vi "Get Default Actor Class Path.vi"(8 "error in (no error)":errorcluster, 11 "Actor Store":refnum<class "Actor Store.lvclass">) -> (0 "error out":errorcluster, 1 "Actor Label":string, 2 "Path String":path, 3 "Actor Store":refnum<class "Actor Store.lvclass">)   [LabVIEW 2023, in "Add Async Methods Actor.lvlib"]
uses:
  Add Async Methods Actor.lvlib
  Classes/Actor Store/Actor Store.lvclass
  <vilib>/Utility/LVLibp/NI_PackedLibraryUtility.lvlib
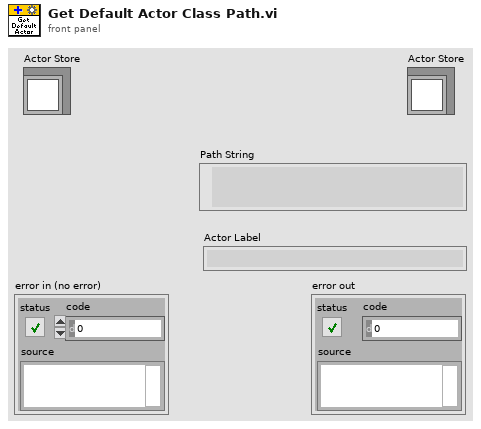
[diagram p1: front panel]
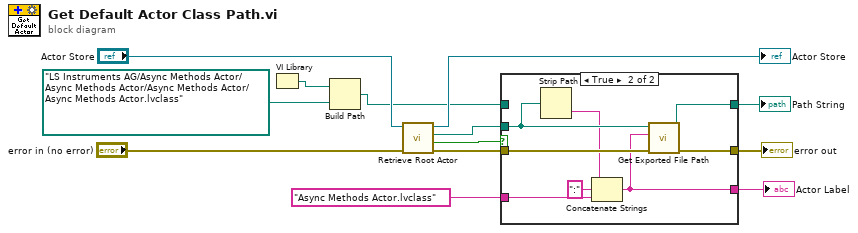
[diagram p0: block diagram]
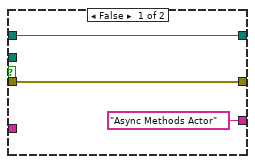
[diagram p2: hidden frame]
diagram:
  n1 = VI Library() -> (path=w4:path)
  n2 = Build Path(base path=w4, name or relative path=path "LS Instruments AG/Async Methods Actor/Async Methods Actor/Async Methods Actor/Async Methods Actor.lvclass") -> (appended path=w2:path)
  n3 = call-dynamic "Retrieve Root Actor.vi"("error in (no error)"="error in (no error)", "Actor Store in"="Actor Store") -> ("error out"=w12:errorcluster, "valid?"=w11:bool, "Root Actor"=w13:path, "Actor Store out"=→"Actor Store":refnum<class "Actor Store.lvclass">)  [unwired: 6 in]
  n4 = case shown="True" w11 {
    tunnel: w12 -> [w16 w24]
    tunnel: [w16 w22] -> w8
    tunnel: w2 -> [w15 _]
    tunnel: [w15 w23] -> w10
    tunnel: w13 -> [_ w20]
    tunnel: "Async Methods Actor.lvclass" ("qualified name") -> [_ w21]
    tunnel: ["Async Methods Actor" w17] -> w7
    frame False {
    }
    frame True {
      n5 = Strip Path(path=w20) -> (name=w19:string)  [unwired: 1 out]
      n6 = Concatenate Strings(w19, ":" ("string"), w21) -> (w17:string)
      n7 = call <vilib>:"Get Exported File Path.vi"("error in (no error)"=w24, "qualified name"=w17, "packed library path"=w20) -> ("error out"=w22:errorcluster, "path"=w23:path)  [unwired: 7 in]
    }
  }
  "error out" <- w8
  "Path String" <- w10
  "Actor Label" <- w7
